vi "Test Overrides Has Mock Class on Dynamic Connectors.vi"(8 "error in (no error)":errorcluster, 11 "Test Case In":refnum<class "_Mock Class Generator Test.lvclass">) -> (0 "error out":errorcluster, 3 "Test Case Out":refnum<class "_Mock Class Generator Test.lvclass">)   [LabVIEW 2020, in "_Mock Class Generator Test.lvclass"]
uses:
  _Mock Class Generator Test.lvclass
  C:/Program Files (x86)/National Instruments/LabVIEW 2020/vi.lib/Astemes/LUnit/Test Case.lvclass
  <vilib>/Astemes/LUnit/Test Case.lvclass/Test Case.ctl
  <vilib>/Astemes/LUnit/Append Pass Result.vi
  <vilib>/Astemes/LUnit/Append Fail Result.vi
  <vilib>/Astemes/LUnit/Run In UI.vi
  <vilib>/Utility/error.llb/Clear Errors.vi
  _Mock Class Generator Test.lvclass/_Mock Class Generator Test.ctl
  source/Scripting/Mock Class Generator/Mock Class Generator.lvclass
  <vilib>/Astemes/LUnit/Test Case.lvclass
  C:/Program Files (x86)/National Instruments/LabVIEW 2020/vi.lib/Astemes/LUnit/LUnit Runnable.lvclass
  C:/git/astemes-lmock/tests/Mock Class Generator Test/_Mock Class Generator Test.lvclass
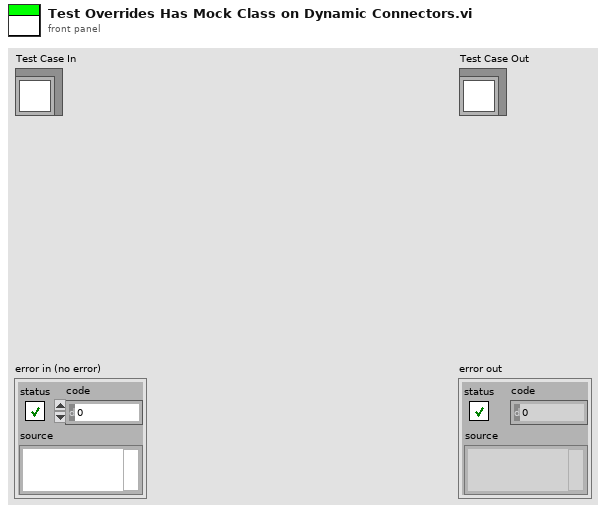
[diagram p1: front panel]
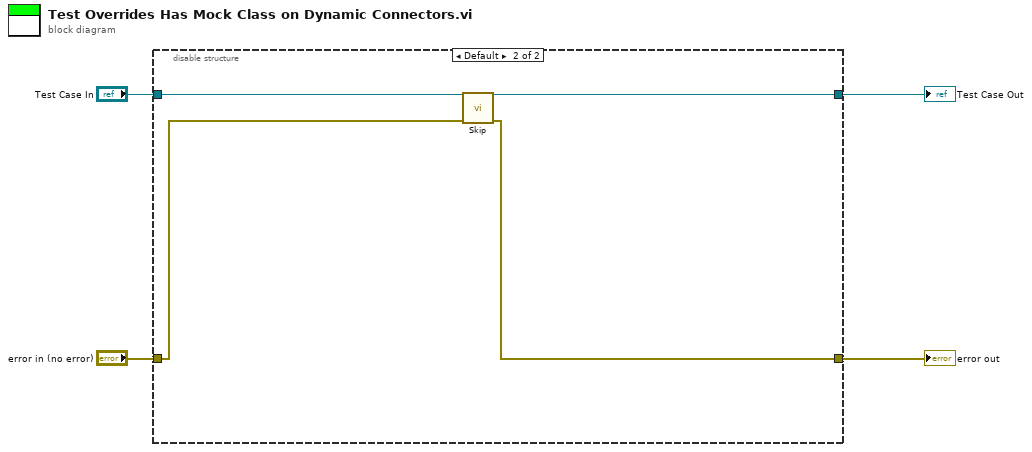
[diagram p0: block diagram]
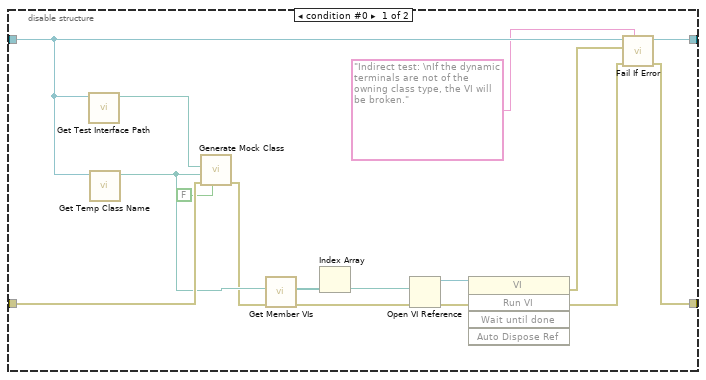
[diagram p2: hidden frame]
diagram:
  n1 = disable-structure shown="Default" {
    disable-tunnel: [w19 w20] -> w4
    disable-tunnel: [w18 w21] -> w3
    disable-tunnel: "Test Case In" -> [w17 w23]
    disable-tunnel: "error in (no error)" -> [w16 w22]
    frame condition #0 {
      n2 = call "Get Test Interface Path.vi"("Mock Class Generator Test in"=w17) -> ("Test Class Path"=w15:path)  [unwired: 10 in]
      n3 = call "Get Temp Class Name.vi"("Mock Class Generator Test in"=w17) -> ("Test Class Path"=w14:path)  [unwired: 10 in]
      n4 = call "Generate Mock Class.vi"("Add to lvproj?"=FALSE, "error in (no error)"=w16, "Destination Class Path"=w14, "Source Class Path"=w15) -> ("error out"=w13:errorcluster)  [unwired: 6 in, 1 out]
      n5 = call "Get Member VIs.vi"("error in (no error)"=w13, "Test Class Path"=w14) -> ("error out"=w12:errorcluster, "Array"=w11:path[])  [unwired: 8 in]
      n6 = Index Array(array=w11) -> (element=w9:path)  [unwired: 1 in]
      n7 = Open VI Reference(vi path=w9, error in (no error)=w12) -> (vi reference=w8:refnum<vi>, error out=w10:errorcluster)  [unwired: 4 in]
      n8 = invoke class="VI" method="Run VI"(reference=w8) -> (error out=w7:errorcluster)  [unwired: 4 in, 4 out]
      n9 = call <vilib>:"Fail If Error.vi"("Description"="Indirect test: \nIf the dynamic terminals are not of the owning class type, the VI will be broken.", "error in (no error)"=w10, "Assert error"=w7, "LUnit Test Case In"=w17) -> ("error out"=w18:errorcluster, "LUnit Test Case Out"=w19:refnum<class "_Mock Class Generator Test.lvclass">)  [unwired: 6 in]
    }
    frame condition #1 (active) {
      n10 = call <vilib>:"Skip.vi"("error in (no error)"=w22, "LUnit Test Case In"=w23) -> ("error out"=w21:errorcluster, "LUnit Test Case Out"=w20:refnum<class "_Mock Class Generator Test.lvclass">)  [unwired: 8 in]
    }
  }
  "error out" <- w3
  "Test Case Out" <- w4
